vi "clear Session Data.vi"(0 "Session in":refnum<class "Execution.lvclass">, 11 "error in":errorcluster) -> (4 "Session out":refnum<class "Execution.lvclass">, 15 "error out":errorcluster)   [LabVIEW 2020, in "TSS.lvlib" / "Execution.lvclass"]
uses:
  Execution.lvclass
  Execution.lvclass/Execution.ctl
  SequenceFile/Typedefs/Session Handle.ctl
  SequenceFile/SequenceFile.lvclass
  VariableContainer/Typedefs/Session Handle.ctl
  VariableContainer/VariableContainer.lvclass
  <userlib>/_Session Fwk/Session - Root.lvclass
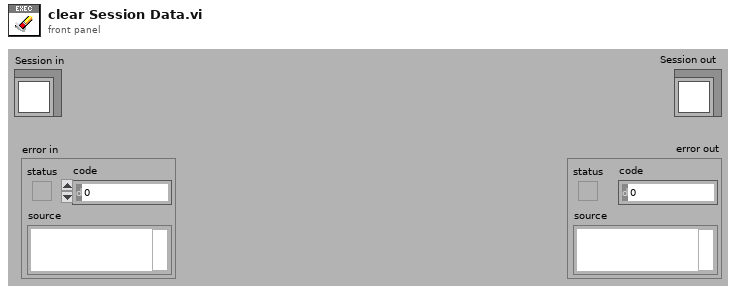
[diagram p1: front panel]
types:
  T1 = typedef "TSS.lvlib/VariableContainer.lvclass/Session Handle.ctl" = refnum<data-value>
  T2 = typedef "TSS.lvlib/SequenceFile.lvclass/Session Handle.ctl" = refnum<data-value>
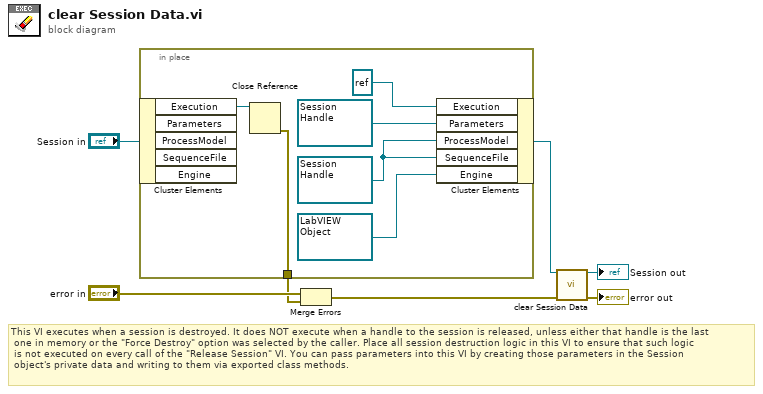
[diagram p0: block diagram]
diagram:
  # "This VI executes when a session is destroyed. It does NOT execute when a handle to the session is released, unless either that handle is the last\n one in memory or the \"Force Destroy\" option was selected by the caller. Place all session destruction logic in this VI to ensure that such logic\n is not executed on every call of the \"Release Session\" VI. You can pass parameters into this VI by creating those parameters in the Session \n object's private data and writing to them via exported class methods."
  n1 = in-place {
    in-place-border: [w9] -> w2
    w12 = T2 refnum ("SequenceFile")
    n2 = in-place-cluster #1("Session in") -> ("Execution"=w13:refnum<k7>)  [unwired: 4 out]
    n3 = Close Reference(reference=w13) -> (error out=w9:errorcluster)  [unwired: 1 in]
    n4 = in-place-cluster #1("Execution"=refnum<k7> refnum, "Parameters"=T1 refnum, "ProcessModel"=w12, "SequenceFile"=w12, "Engine"=refnum<data-value> refnum) -> (w4:refnum<class "Execution.lvclass">)
  }
  n5 = Merge Errors("error in", w2) -> (w3:errorcluster)
  n6 = call-parent "clear Session Data.vi"("OBJ - Measurement Session in"=w4, "error in"=w3) -> ("OBJ - Measurement Session out"=→"Session out":refnum<class "Execution.lvclass">, "error out"=→"error out":errorcluster)  [unwired: 12 in]
